vi "VIH Utility - DEV - Get DevTime Utility VIs Folder.vi"(8 "error in":errorcluster, 10 "Utility VI Name":string) -> (0 "error out":errorcluster, 2 "Utility VIs Path":path, 3 "Utility VIs Folder":path)   [LabVIEW 2014]
doc: "::: VI Helpeks :::\nCopyright (c) 2000-2026 Konstantin Shifershteyn. All rights reserved."
panel:
  # "VI Helpeks\nCopyright (c) 2012-2026 Konstantin Shifershteyn"
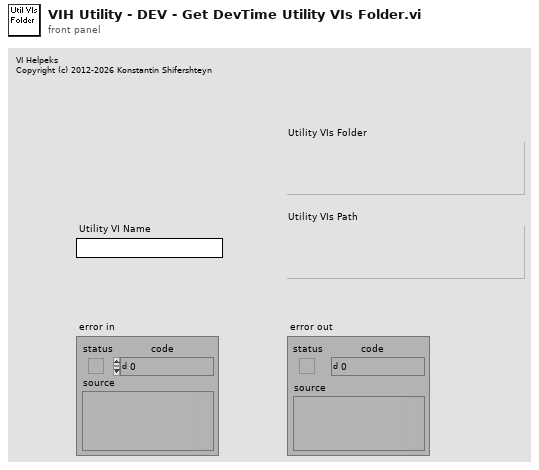
[diagram p1: front panel]
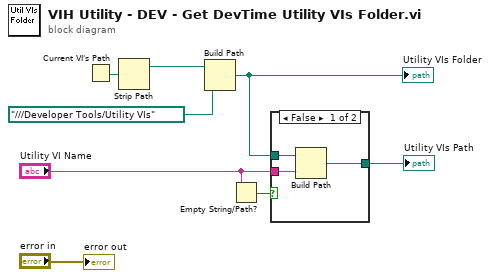
[diagram p0: block diagram]
diagram:
  n1 = Current VI's Path() -> (path=w8:path)
  n2 = Strip Path(path=w8) -> (stripped path=w5:path)  [unwired: 1 out]
  n3 = Build Path(base path=w5, name or relative path=path "../../../Developer Tools/Utility VIs") -> (appended path=w4:path)
  "Utility VIs Folder" <- w4
  n4 = Empty String/Path?(string/path="Utility VI Name") -> (empty?=w2:bool)
  n5 = case shown="False" w2 {
    tunnel: "Utility VI Name" -> [w11 _]
    tunnel: [w10 _] -> w6
    tunnel: w4 -> [w9 _]
    frame False {
      n6 = Build Path(base path=w9, name or relative path=w11) -> (appended path=w10:path)
    }
    frame True {
    }
  }
  "Utility VIs Path" <- w6
  "error out" <- "error in"
